vi "test-Chain mode.vi"(8 "error in (no error)":errorcluster, 11 "TestCase in":refnum<class "testcase-CSMAttributes.lvclass">) -> (0 "error out":errorcluster, 3 "TestCase out":refnum<class "testcase-CSMAttributes.lvclass">)   [LabVIEW 2017, in "testcase-CSMAttributes.lvclass"]
uses:
  testcase-CSMAttributes.lvclass
  6faf3dd6-bbe3-43e6-ac0e-6a595a4bbb73.vi
  eea55257-98dc-4069-a2fc-7f3abec53d34.vi
  654a1434-e049-45b7-bbe1-b3daff27deed.vi
  232dea5e-886f-41b8-bb39-dacd9565842e.vi
  d39486ea-fbfe-4c2b-b0ae-85d31efdfc25.vi
  4fbfc3b2-4ab6-4b17-950e-362f3a1418f9.vi
  eb53d3db-f5cc-4d50-900d-3a282fe3921b.vi
  d3eb8ef0-7d19-473b-ace2-fe9805f10b86.vi
  src/user.lib/_NEVSTOP/Communicable State Machine(CSM)/AdvanceAPI/CSM - Set Module Attribute.vi
  src/user.lib/_NEVSTOP/Communicable State Machine(CSM)/AdvanceAPI/CSM - Get Module Attribute.vi
  src/user.lib/_NEVSTOP/Communicable State Machine(CSM)/Communicable State Machine.lvlib
  <vilib>/addons/_JKI Toolkits/VI Tester/TestCase.llb/TestCase.lvclass
  C:/Program Files (x86)/National Instruments/LabVIEW 2017/vi.lib/addons/_JKI Toolkits/VI Tester/TestCase.llb/TestCase.lvclass
panel:
  out "error out":errorcluster
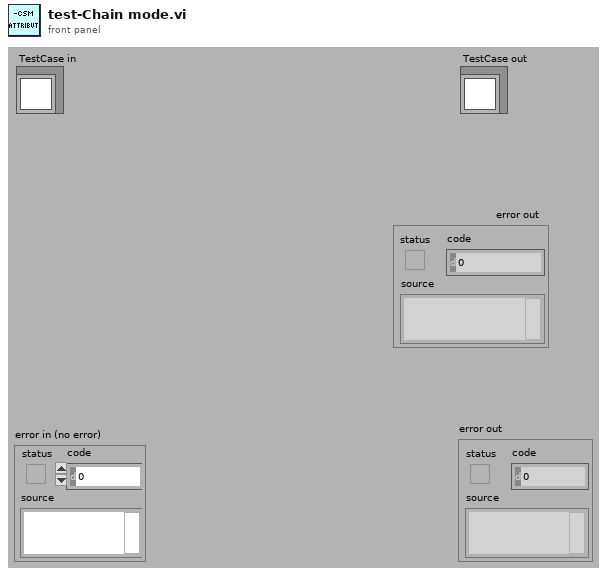
[diagram p1: front panel]
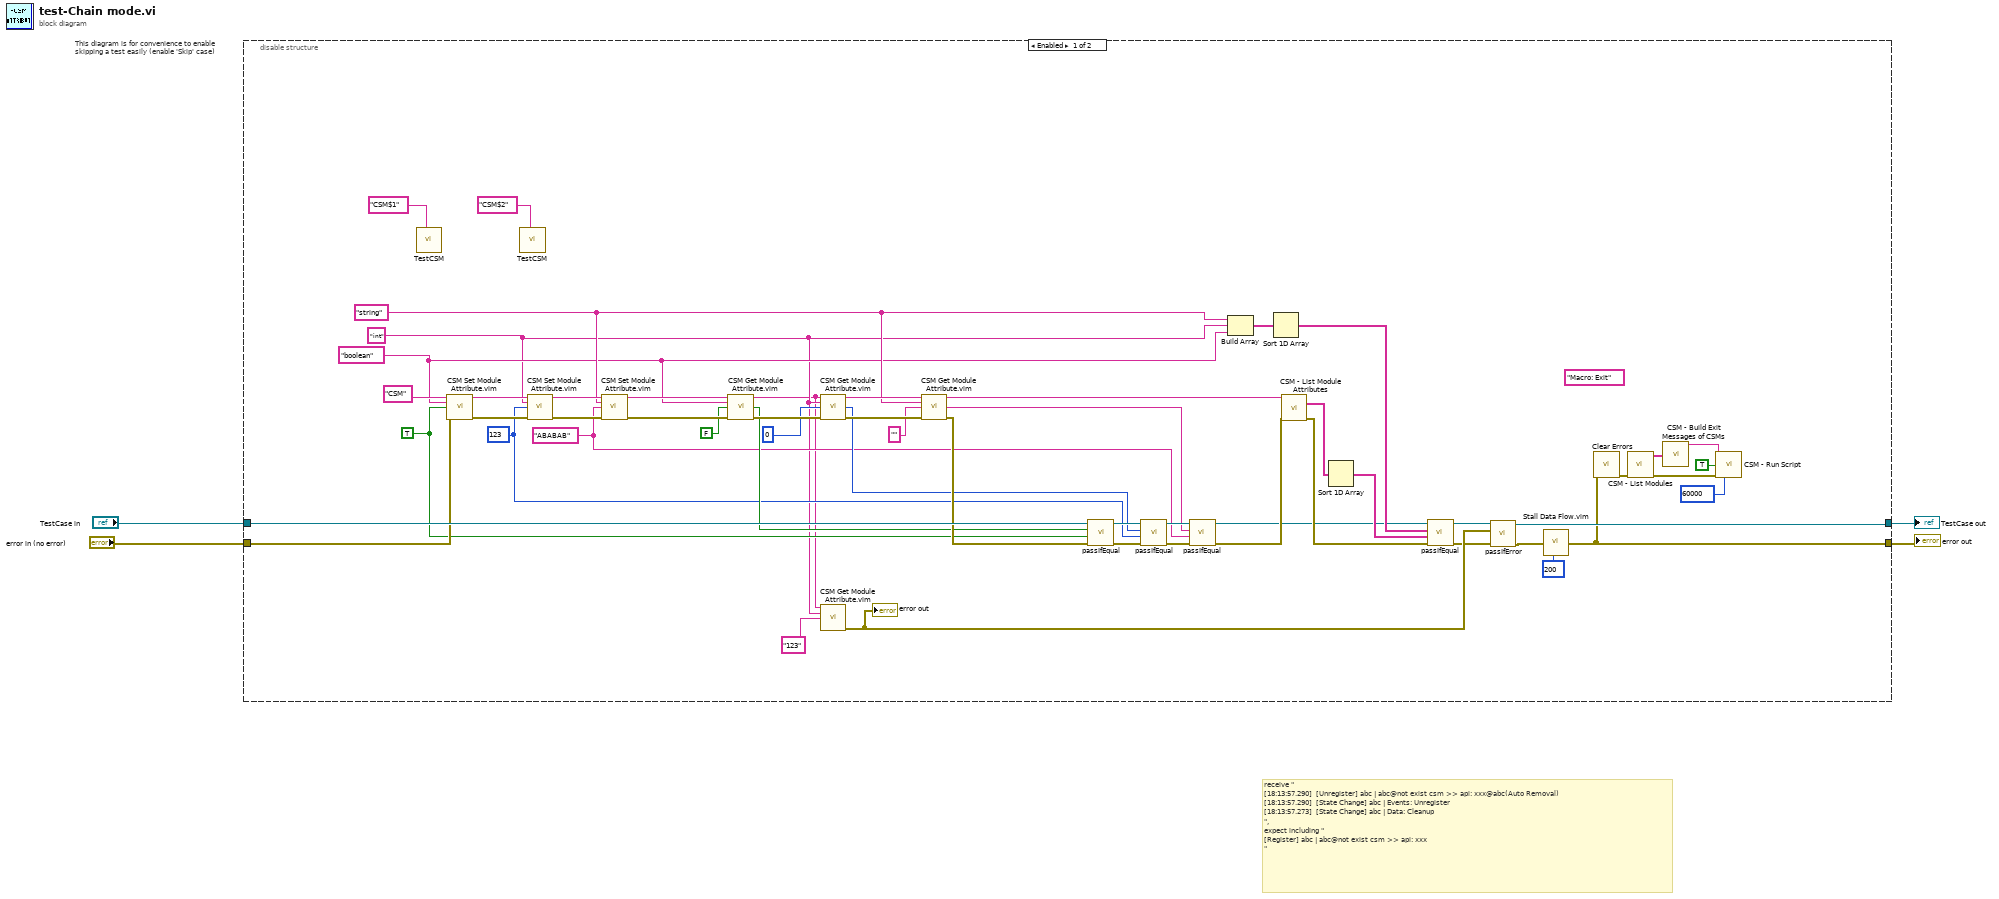
[diagram p0: block diagram]
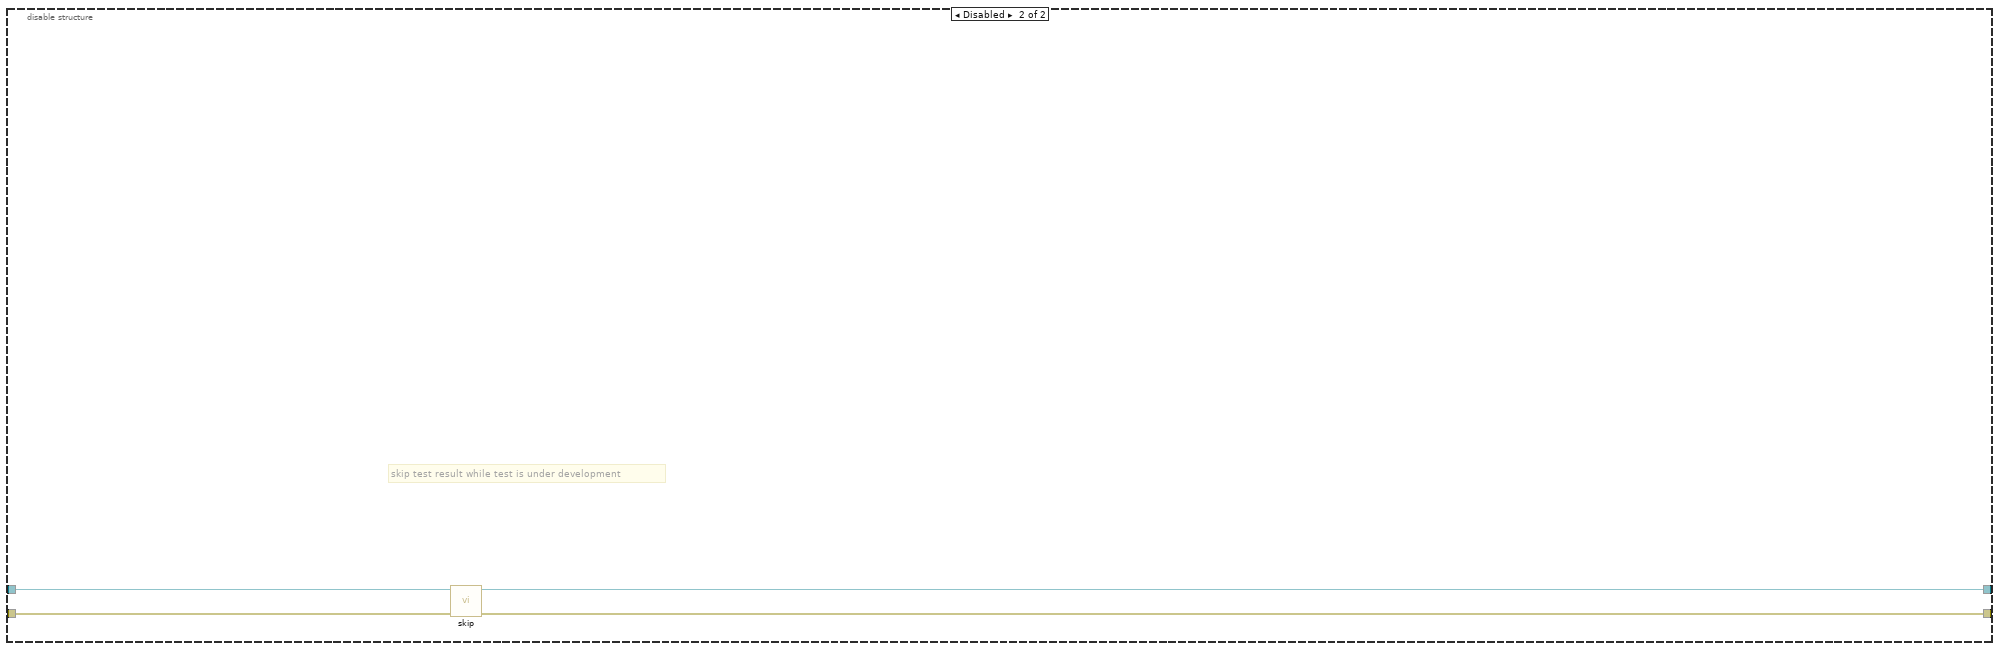
[diagram p2: hidden frame]
diagram:
  # "receive \"\n[18:13:57.290]  [Unregister] abc | abc@not exist csm >> api: xxx@abc(Auto Removal)\n[18:13:57.290]  [State Change] abc | Events: Unregister\n[18:13:57.273]  [State Change] abc | Data: Cleanup\n\", \nexpect including \"\n[Register] abc | abc@not exist csm >> api: xxx\n\""
  n1 = disable-structure "This diagram is for convenience to enable skipping a test easily (enable 'Skip' case)" shown="Enabled" {
    disable-tunnel: "TestCase in" -> [w58 w62]
    disable-tunnel: [w14 w60] -> w1
    disable-tunnel: [w8 w61] -> w3
    disable-tunnel: "error in (no error)" -> [w57 w59]
    frame Enabled {
      (unwired) "Macro: Exit" ("State")
      w33 = "ABABAB" ("Attribute")
      w29 = "string" ("Attribute")
      w37 = 123
      w20 = "int" ("Attribute")
      w42 = TRUE
      w28 = "boolean" ("Attribute")
      n2 = call "TestCSM.vi"("Name (\"\" to Use UUID)"="CSM$1" ("Name (\"\" to Use UUID)")) -> ()  [unwired: 11 in]
      n3 = call "CSM Set Module Attribute.vim"("CSM Name"="CSM" ("Name (\"\" to Use UUID)"), "Attribute"=w28, "Value"=w42, "Error In"=w57) -> ("CSM Name (Dup)"=w53:string, "error out"=w55:errorcluster)  [unwired: 8 in, 2 out]
      n4 = call "TestCSM.vi"("Name (\"\" to Use UUID)"="CSM$2" ("Name (\"\" to Use UUID)")) -> ()  [unwired: 11 in]
      n5 = call "CSM Set Module Attribute.vim"("CSM Name"=w53, "Attribute"=w20, "Value"=w37, "Error In"=w55) -> ("CSM Name (Dup)"=w52:string, "error out"=w54:errorcluster)  [unwired: 8 in, 2 out]
      n6 = call "CSM Set Module Attribute.vim"("CSM Name"=w52, "Attribute"=w29, "Value"=w33, "Error In"=w54) -> ("CSM Name (Dup)"=w50:string, "error out"=w51:errorcluster)  [unwired: 8 in, 2 out]
      n7 = call "CSM Get Module Attribute.vim"("CSM Name"=w50, "Attribute"=w28, "Default Value (Empty Variant)"=FALSE, "Error In"=w51) -> ("CSM Name (Dup)"=w19:string, "Value"=w41:bool, "error out"=w49:errorcluster)  [unwired: 7 in, 2 out]
      n8 = call "CSM Get Module Attribute.vim"("CSM Name"=w19, "Attribute"=w20, "Default Value (Empty Variant)"=0, "Error In"=w49) -> ("CSM Name (Dup)"=w48:string, "Value"=w38:i32, "error out"=w47:errorcluster)  [unwired: 7 in, 2 out]
      n9 = call "CSM Get Module Attribute.vim"("CSM Name"=w19, "Attribute"=w20, "Default Value (Empty Variant)"="123") -> ("error out"=w17:errorcluster)  [unwired: 8 in, 4 out]
      "error out" <- w17
      n10 = call "CSM Get Module Attribute.vim"("CSM Name"=w48, "Attribute"=w29, "Default Value (Empty Variant)"="" ("Attribute"), "Error In"=w47) -> ("CSM Name (Dup)"=w32:string, "Value"=w34:string, "error out"=w43:errorcluster)  [unwired: 7 in, 2 out]
      n11 = call-dynamic "passIfEqual.vi"("error in (no error)"=w43, "y"=w42, "x"=w41, "TestCase in"=w58) -> ("error out"=w39:errorcluster, "TestCase out"=w40:refnum<class "testcase-CSMAttributes.lvclass">)  [unwired: 6 in]
      n12 = call-dynamic "passIfEqual.vi"("error in (no error)"=w39, "y"=w37, "x"=w38, "TestCase in"=w40) -> ("error out"=w35:errorcluster, "TestCase out"=w36:refnum<class "testcase-CSMAttributes.lvclass">)  [unwired: 6 in]
      n13 = call-dynamic "passIfEqual.vi"("error in (no error)"=w35, "y"=w33, "x"=w34, "TestCase in"=w36) -> ("error out"=w31:errorcluster, "TestCase out"=w23:refnum<class "testcase-CSMAttributes.lvclass">)  [unwired: 6 in]
      n14 = Build Array(w29, w20, w28) -> (w27:string[])
      n15 = Sort 1D Array(array=w27) -> (sorted array=w24:string[])
      n16 = call "CSM - List Module Attributes.vi"("CSM Name"=w32, "Error In"=w31) -> ("Attributes"=w26:string[], "error out"=w30:errorcluster)  [unwired: 9 in, 3 out]
      n17 = Sort 1D Array(array=w26) -> (sorted array=w25:string[])
      n18 = call-dynamic "passIfEqual.vi"("error in (no error)"=w30, "y"=w25, "x"=w24, "TestCase in"=w23) -> ("error out"=w16:errorcluster, "TestCase out"=w18:refnum<class "testcase-CSMAttributes.lvclass">)  [unwired: 6 in]
      n19 = call-dynamic "passIfError.vi"("error in (no error)"=w16, "error"=w17, "TestCase in"=w18) -> ("error out"=w15:errorcluster, "TestCase out"=w14:refnum<class "testcase-CSMAttributes.lvclass">)  [unwired: 7 in]
      n20 = call "Stall Data Flow.vim"("value in"=w15, "milliseconds to wait"=u32 200) -> ("value out"=w8:errorcluster)  [unwired: 1 out]
      n21 = call <vilib>:"Clear Errors.vi"("error in (no error)"=w8) -> ("error out"=w22:errorcluster)  [unwired: 5 in, 1 out]
      n22 = call "CSM - List Modules.vi"("Error In"=w22) -> ("error out"=w12:errorcluster, "Module Names"=w11:string[])  [unwired: 9 in]
      n23 = call "CSM - Build Exit Messages of CSMs.vi"("CSMs"=w11) -> ("States"=w9:string)  [unwired: 14 in]
      n24 = call "CSM - Run Script.vi"("CSM Scripts"=w9, "Continue If Error? (F)"=TRUE ("Continue If Error?(F)"), "error in (no error)"=w12, "Response Timeout (-2 Using Global Settings)"=60000) -> ()  [unwired: 9 in, 3 out]
    }
    frame Disabled {
      # "skip test result while test is under development"
      n25 = call <vilib>:"skip.vi"("error in (no error)"=w59, "TestCase in"=w62) -> ("error out"=w61:errorcluster, "TestCase out"=w60:refnum<class "testcase-CSMAttributes.lvclass">)  [unwired: 8 in]
    }
  }
  "error out" <- w3
  "TestCase out" <- w1
